vi "Setup TS.vi"(8 "error in":errorcluster, 11 "Test Stand in":refnum<class "Heat Flow Test Stand.lvclass">) -> (0 "error out":errorcluster, 3 "Test Stand out":refnum<class "Heat Flow Test Stand.lvclass">)   [LabVIEW 2019, in "Test Stands.lvlib" / "Heat Flow Test Stand.lvclass"]
uses:
  Heat Flow Test Stand.lvclass
  C:/Users/krio/Documents/LV_Projects/test-stand/App/Generic Test Stand/Generic Test Stand.lvclass
  DAC/Heat Flow/HeatFlow AIV/DAC HeatFlow AIV.lvclass
  C:/Users/krio/Documents/LV_Projects/test-stand/App/DAC/DAC.lvclass
  DAC/Heat Flow/HeatFlow AOV/DAC HeatFlow AOV.lvclass
  DAC/Heat Flow/TEG Temp/DAC TEG Temp.lvclass
  DAC/Heat Flow/RTD Temp/DAC RTD Temp.lvclass
  DAC/DAC.lvclass/DAC.ctl
  Generic Test Stand/Generic Test Stand.lvclass/Generic Test Stand.ctl
  Heat Flow Test Stand.lvclass/Heat Flow Test Stand.ctl
  Generic Test Stand/Generic Test Stand.lvclass
  DAC/DAC.lvclass
  DAC/Heat Flow/HeatFlow Load dU/DAC HeatFlow Load dU.lvclass
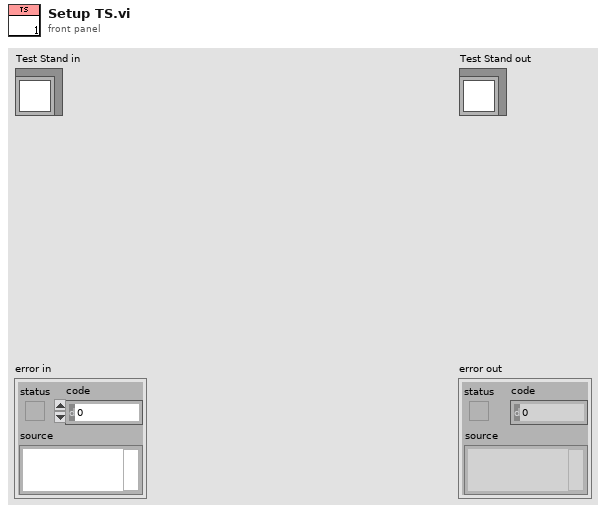
[diagram p1: front panel]
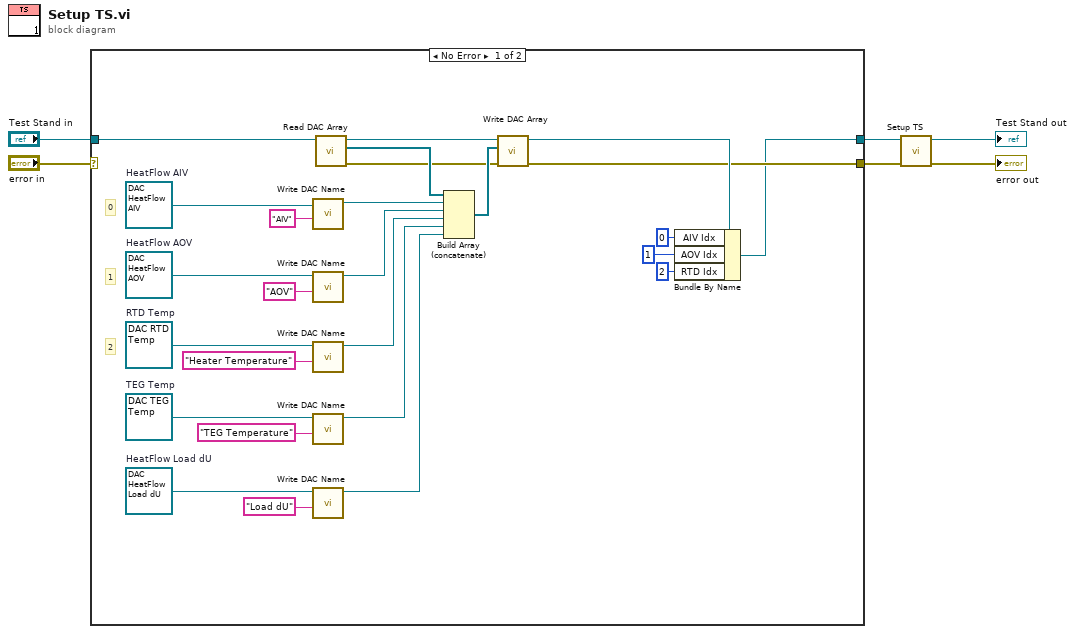
[diagram p0: block diagram]
diagram:
  n1 = case shown="No Error" "error in" {
    selector: "error in" -> [_ w33]
    tunnel: "Test Stand in" -> [w32 w34]
    tunnel: [w22 w34] -> w2
    tunnel: [w25 w33] -> w1
    frame No Error {
      w8 = refnum<class "DAC HeatFlow Load dU.lvclass"> refnum  # HeatFlow Load dU
      w12 = refnum<class "DAC RTD Temp.lvclass"> refnum  # RTD Temp
      w13 = refnum<class "DAC TEG Temp.lvclass"> refnum  # TEG Temp
      w20 = refnum<class "DAC HeatFlow AOV.lvclass"> refnum  # HeatFlow AOV
      w23 = refnum<class "DAC HeatFlow AIV.lvclass"> refnum  # HeatFlow AIV
      # "2"
      # "1"
      # "0"
      n2 = call "Write DAC Name.vi"("DAC Name"="AIV", "DAC in"=w23) -> ("DAC out"=w24:refnum<class "DAC HeatFlow AIV.lvclass">)  [unwired: 8 in, 1 out]
      n3 = call "Write DAC Name.vi"("DAC Name"="AOV", "DAC in"=w20) -> ("DAC out"=w19:refnum<class "DAC HeatFlow AOV.lvclass">)  [unwired: 8 in, 1 out]
      n4 = call "Write DAC Name.vi"("DAC Name"="Heater Temperature", "DAC in"=w12) -> ("DAC out"=w18:refnum<class "DAC RTD Temp.lvclass">)  [unwired: 8 in, 1 out]
      n5 = call "Write DAC Name.vi"("DAC Name"="TEG Temperature", "DAC in"=w13) -> ("DAC out"=w11:refnum<class "DAC TEG Temp.lvclass">)  [unwired: 8 in, 1 out]
      n6 = call "Write DAC Name.vi"("DAC Name"="Load dU", "DAC in"=w8) -> ("DAC out"=w7:refnum<class "DAC HeatFlow Load dU.lvclass">)  [unwired: 8 in, 1 out]
      n7 = call "Read DAC Array.vi"("Generic Test Stand in"=w32) -> ("error out"=w28:errorcluster, "DAC Array"=w31:refnum<class "DAC.lvclass">[], "Generic Test Stand out"=w30:refnum<class "Heat Flow Test Stand.lvclass">)  [unwired: 8 in]
      n8 = Build Array (concatenate)(w31, w24, w19, w18, w11, w7) -> (w29:refnum<class "DAC.lvclass">[])
      n9 = call "Write DAC Array.vi"("error in (no error)"=w28, "DAC Array"=w29, "Generic Test Stand in"=w30) -> ("error out"=w25:errorcluster, "Generic Test Stand out"=w26:refnum<class "Heat Flow Test Stand.lvclass">)  [unwired: 7 in]
      n10 = Bundle By Name(cluster=w26, "AIV Idx"=0, "AOV Idx"=1, "RTD Idx"=2) -> (w22:refnum<class "Heat Flow Test Stand.lvclass">)
    }
    frame Error {
    }
  }
  n11 = call-parent "Setup TS.vi"("error in (no error)"=w1, "Generic Test Stand in"=w2) -> ("error out"=→"error out":errorcluster, "Generic Test Stand out"=→"Test Stand out":refnum<class "Heat Flow Test Stand.lvclass">)  [unwired: 8 in]
